vi "Get Port.vi"(8 "error in (no error)":errorcluster caption="에러 입력(에러 없음)", 11 "CE RF Switch Box 입력":refnum<class "CE RF Switch Box.lvclass">) -> (0 "error out":errorcluster caption="에러 출력", 1 "Filter path":T1, 2 "Input path":T2, 3 "CE RF Switch Box 출력":refnum<class "CE RF Switch Box.lvclass">)   [LabVIEW 2023, in "RF Switch Box.lvlib" / "CE RF Switch Box.lvclass"]
uses:
  CE RF Switch Box.lvclass
  Type Definition/Input path.ctl
  Type Definition/Filter path.ctl
  CE RF Switch Box.lvclass/CE RF Switch Box.ctl
  RF Switch Box.lvlib
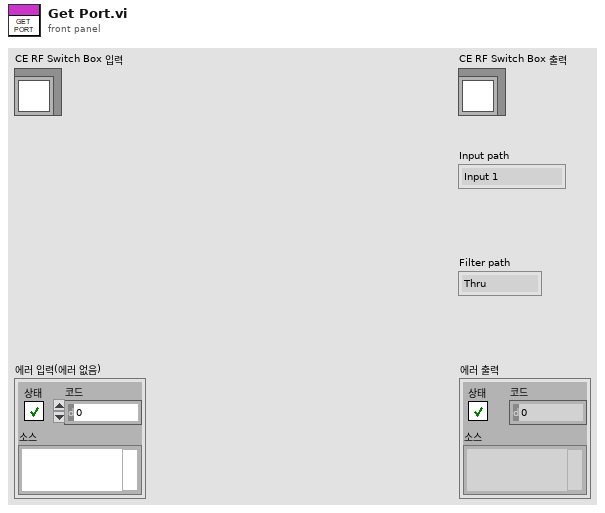
[diagram p1: front panel]
types:
  T1 = typedef "RF Switch Box.lvlib/Filter path.ctl" = enum16{"Thru", "Direct Amp", "1G HPF", "3G HPF", "7G HPF", "6G HPF", "port 1", "port 2", "port 3", "port 4", "port 5", "port 6", "port 7", "port 8", "port 9", "port 10", "port 11", "port 12", "port 13", "port 14", "port 15", "port 16", "port 17", "port 18"}
  T2 = typedef "RF Switch Box.lvlib/Input path.ctl" = enum16{"Input 1", "Input 2", "Input 3"}
  T3 = enum16{"Standard", "Buffered", "CRLF", "Immediate"}
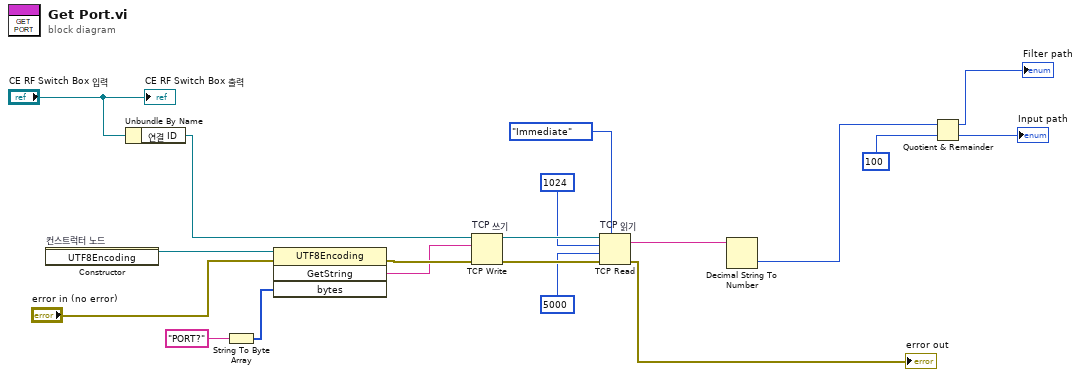
[diagram p0: block diagram]
diagram:
  n1 = constructor on="컨스트럭터 노드" class="UTF8Encoding"() -> (reference out=w18:refnum<k24>)  [unwired: 3 in, 2 out]
  n2 = Unbundle By Name("CE RF Switch Box 입력") -> ("연결 ID"=w10:refnum<k5>)
  n3 = String To Byte Array(string="PORT?" ("데이터 입력")) -> (unsigned byte array=w16:u8[])
  n4 = invoke class="UTF8Encoding" method="GetString"(reference=w18, error in="error in (no error)", "bytes"=w16) -> (error out=w11:errorcluster, "GetString"=w9:string)  [unwired: 1 in, 2 out]
  n5 = TCP Write "TCP 쓰기"(connection ID=w10, data in=w9, error in (no error)=w11) -> (connection ID out=w14:refnum<k5>, error out=w15:errorcluster)  [unwired: 1 in, 1 out]
  n6 = TCP Read "TCP 읽기"(connection ID=w14, bytes to read=1024 ("읽을 바이트"), error in (no error)=w15, 7:T3."Immediate" ("모드(standard)"), 9:5000 ("타임아웃 ms (25000)")) -> (data out=w6:string, error out=→"error out":errorcluster)  [unwired: 1 out]
  n7 = Decimal String To Number(string=w6) -> (number=w5:i32)  [unwired: 2 in, 1 out]
  n8 = Quotient & Remainder(x=w5, y=100) -> (x-y*floor(x/y)=→"Filter path":i32, floor(x/y)=→"Input path":i32)
  "CE RF Switch Box 출력" <- "CE RF Switch Box 입력"
